vi "GetConfigurationType.vi"(8 "error in (no error)":errorcluster, 11 "object in":refnum<class "DIO_Channel.lvclass">) -> (0 "error out":errorcluster, 2 "Configuration":refnum<class "Configuration.lvclass">, 3 "object out":refnum<class "DIO_Channel.lvclass">)   [LabVIEW 2021]
doc: "Gets the Configuration to use"
uses:
  DIO_Channel.lvclass
  Generic Channel/Configuration/Configuration.lvclass
  DIO-Configuration_class/DIO-Configuration.lvclass
  C:/Users/averna/Documents/LV Gym DEMO/Factory Pattern/Generic Channel/Configuration/Configuration.lvclass
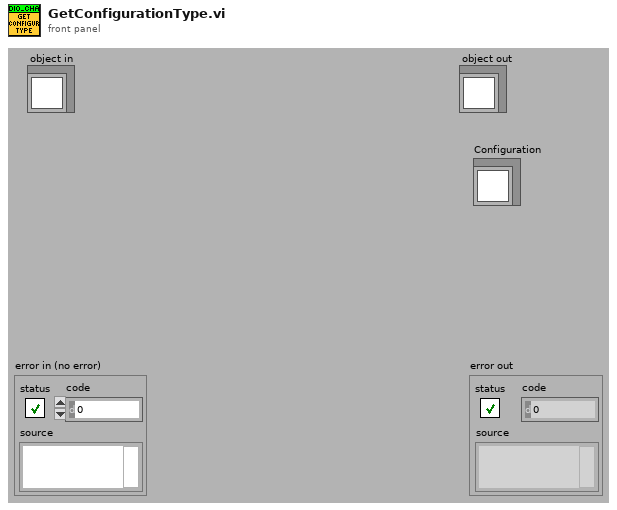
[diagram p1: front panel]
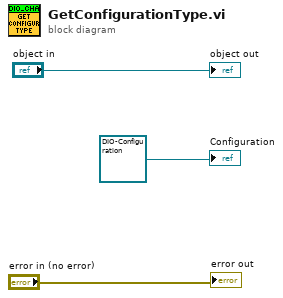
[diagram p0: block diagram]
diagram:
  "error out" <- "error in (no error)"
  "object out" <- "object in"
  "Configuration" <- refnum<class "DIO-Configuration.lvclass"> refnum ("Template-Channels.lvlib:Template_CFG")
